vi "wait Command Interval.vi"(8 "error in (no error)":errorcluster, 11 "NR in":refnum<class "NR.lvclass">) -> (0 "error out":errorcluster, 3 "NR out":refnum<class "NR.lvclass">)   [LabVIEW 2023, in "ANRITSU Call Box.lvlib" / "NR.lvclass"]
uses:
  NR.lvclass
  NR.lvclass/NR.ctl
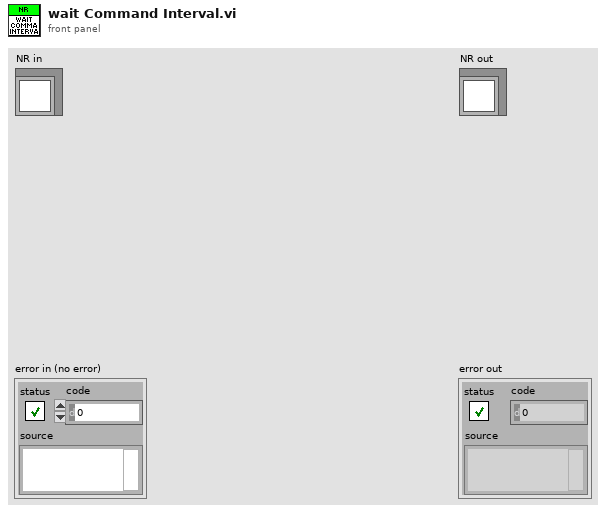
[diagram p1: front panel]
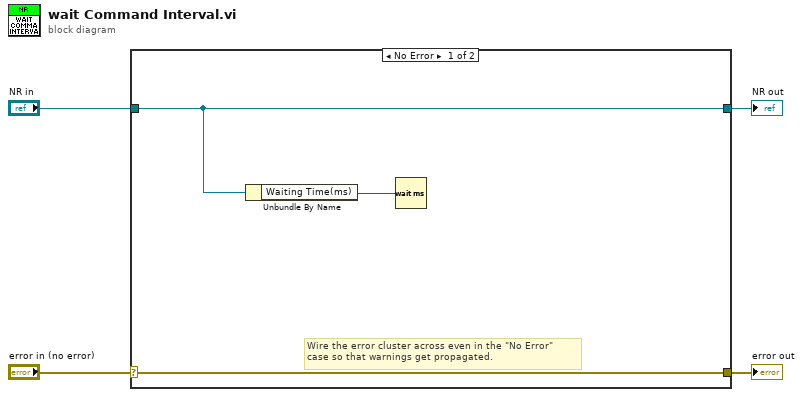
[diagram p0: block diagram]
diagram:
  n1 = case shown="No Error" "error in (no error)" {
    selector: "error in (no error)" -> [w7 w9]
    tunnel: [w7 w9] -> w3
    tunnel: [w6 w8] -> w1
    tunnel: "NR in" -> [w6 w8]
    frame No Error {
      # "Wire the error cluster across even in the \"No Error\"\ncase so that warnings get propagated."
      n2 = Unbundle By Name(w6) -> ("Waiting Time(ms)"=w5:u32)
      n3 = Wait (ms)(milliseconds to wait=w5) -> ()  [unwired: 1 out]
    }
    frame Error {
    }
  }
  "error out" <- w3
  "NR out" <- w1
